vi "保持时间脚本.vi"(8 "4-wire":bool, 11 "保持时间":T1={"V"=0.1, "limit I"=0.01, "T"=10000.0, "ΔT"=1.0, "NPLC"=1.0} {"ΔT" min=0.5 max=100.0 step=0.1 format="%#_6ps"; "T" min=10.0 max=4294000.0 step=1.0 format="%#_6ps"; "NPLC" min=1.0 max=20.0 step=1.0; "limit I" min=1e-08 max=3.0 format="%#_6pA"; "V" min=-40.0 max=40.0 format="%#_6pV"}) -> (3 "Script":string)   [LabVIEW 2020, in "功能选择.xctl"]
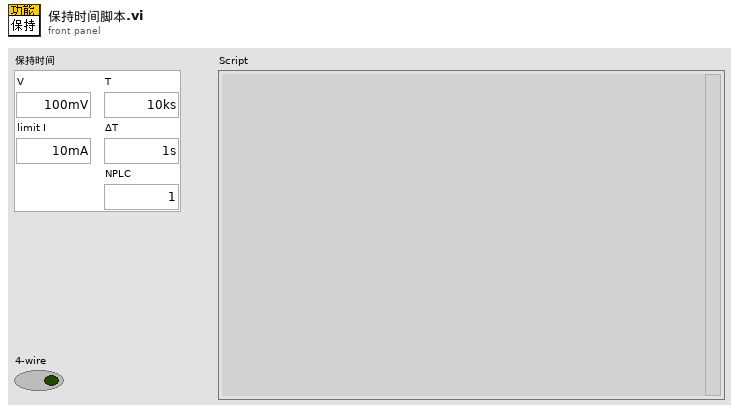
[diagram p1: front panel]
types:
  T1 = typedef "功能选择.xctl/保持时间.ctl" = cluster{"V":dbl, "limit I":dbl, "T":dbl, "ΔT":dbl, "NPLC":dbl}
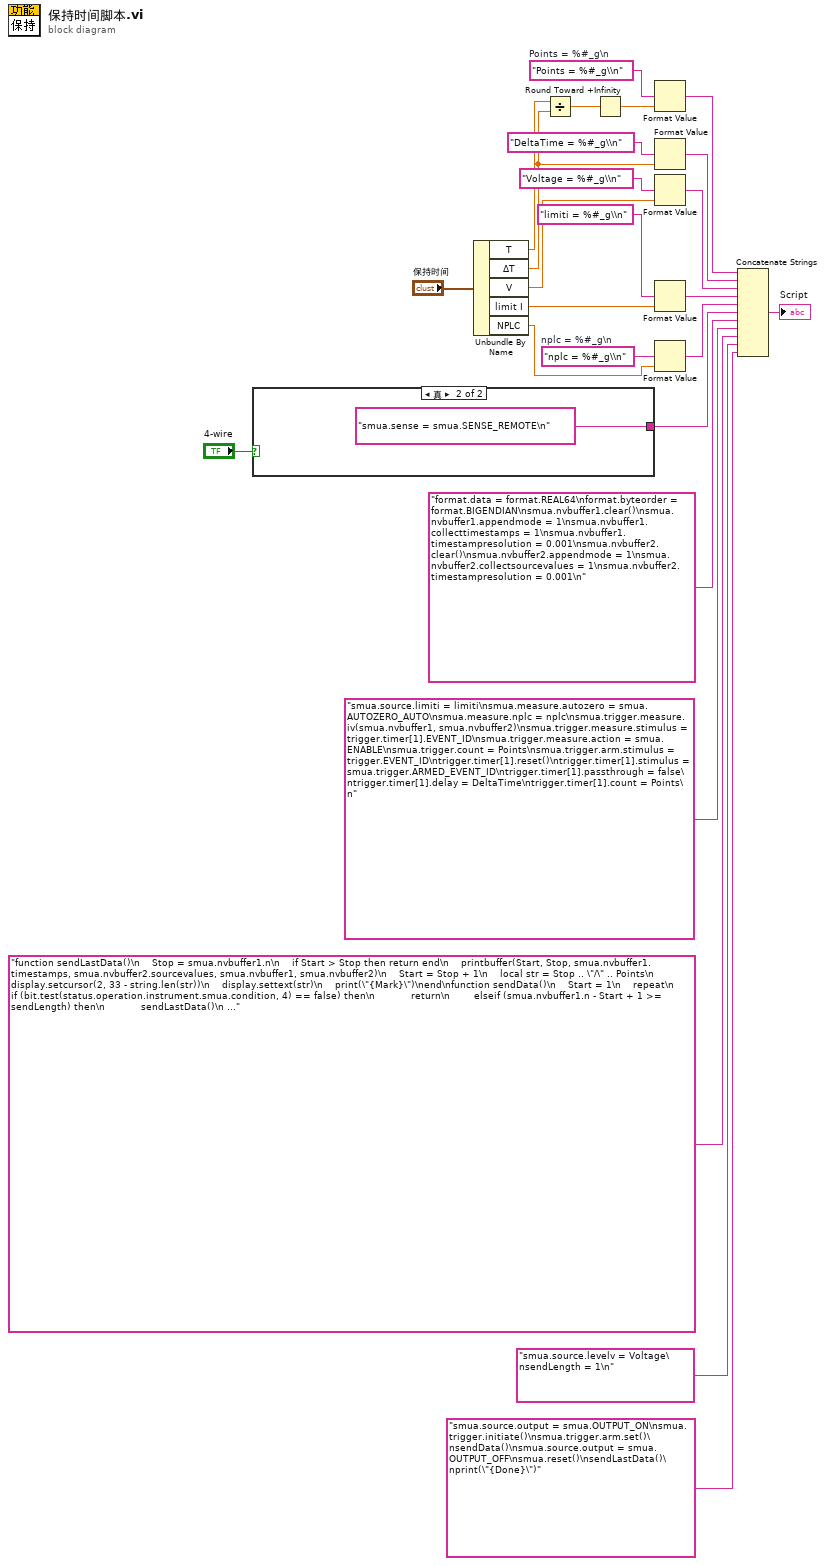
[diagram p0: block diagram]
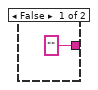
[diagram p2: hidden frame]
diagram:
  w17 = "nplc = %#_g\\n"  # nplc = %#_g\n
  w16 = "Points = %#_g\\n"  # Points = %#_g\n
  n1 = case shown="真" "4-wire" {
    tunnel: ["" "smua.sense = smua.SENSE_REMOTE\n"] -> w6
    frame False {
    }
    frame True {
    }
  }
  n2 = Unbundle By Name("保持时间") -> ("T"=w14:dbl, "ΔT"=w13:dbl, "V"=w11:dbl, "limit I"=w10:dbl, "NPLC"=w7:dbl)
  n3 = Divide(x=w14, y=w13) -> (x/y=w15:dbl)
  n4 = Round Toward +Infinity(x=w15) -> (ceil(x): smallest int >= x=w12:dbl)
  n5 = Format Value(format string=w16, value (0)=w12) -> (output string=w25:string)  [unwired: 1 in]
  n6 = Format Value(format string="DeltaTime = %#_g\\n" ("格式字符串"), value (0)=w13) -> (output string=w23:string)  [unwired: 1 in]
  n7 = Format Value(format string="Voltage = %#_g\\n" ("格式字符串"), value (0)=w11) -> (output string=w9:string)  [unwired: 1 in]
  n8 = Format Value(format string="limiti = %#_g\\n" ("格式字符串"), value (0)=w10) -> (output string=w8:string)  [unwired: 1 in]
  n9 = Format Value(format string=w17, value (0)=w7) -> (output string=w22:string)  [unwired: 1 in]
  n10 = Concatenate Strings(w25, w23, w9, w8, w22, w6, "format.data = format.REAL64\nformat.byteorder = format.BIGENDIAN\nsmua.nvbuffer1.clear()\nsmua.nvbuffer1.appendmode = 1\nsmua.nvbuffer1.collecttimestamps = 1\nsmua.nvbuffer1.timestampresolution = 0.001\nsmua.nvbuffer2.clear()\nsmua.nvbuffer2.appendmode = 1\nsmua.nvbuffer2.collectsourcevalues = 1\nsmua.nvbuffer2.timestampresolution = 0.001\n", "smua.source.limiti = limiti\nsmua.measure.autozero = smua.AUTOZERO_AUTO\nsmua.measure.nplc = nplc\nsmua.trigger.measure.iv(smua.nvbuffer1, smua.nvbuffer2)\nsmua.trigger.measure.stimulus = trigger.timer[1].EVENT_ID\nsmua.trigger.measure.action = smua.ENABLE\nsmua.trigger.count = Points\nsmua.trigger.arm.stimulus = trigger.EVENT_ID\ntrigger.timer[1].reset()\ntrigger.timer[1].stimulus = smua.trigger.ARMED_EVENT_ID\ntrigger.timer[1].passthrough = false\ntrigger.timer[1].delay = DeltaTime\ntrigger.timer[1].count = Points\n", "function sendLastData()\n    Stop = smua.nvbuffer1.n\n    if Start > Stop then return end\n    printbuffer(Start, Stop, smua.nvbuffer1.timestamps, smua.nvbuffer2.sourcevalues, smua.nvbuffer1, smua.nvbuffer2)\n    Start = Stop + 1\n    local str = Stop .. \"/\" .. Points\n    display.setcursor(2, 33 - string.len(str))\n    display.settext(str)\n    print(\"{Mark}\")\nend\nfunction sendData()\n    Start = 1\n    repeat\n        if (bit.test(status.operation.instrument.smua.condition, 4) == false) then\n            return\n        elseif (smua.nvbuffer1.n - Start + 1 >= sendLength) then\n            sendLastData()\n        end\n        delay(DeltaTime)\n    until (false)\nend\n", "smua.source.levelv = Voltage\nsendLength = 1\n", "smua.source.output = smua.OUTPUT_ON\nsmua.trigger.initiate()\nsmua.trigger.arm.set()\nsendData()\nsmua.source.output = smua.OUTPUT_OFF\nsmua.reset()\nsendLastData()\nprint(\"{Done}\")") -> (→"Script":string)
